vi "MES_Post.vi"(8 "error in (no error)":errorcluster, 10 "Body":string, 11 "Path":string) -> (0 "error out":errorcluster, 1 "Response":string, 2 "Code":string, 3 "MES OK":bool)   [LabVIEW 2018]
uses:
  <vilib>/httpClient/LabVIEWHTTPClient.lvlib
  <vilib>/httpClient/POSTBuffer.vi
  <vilib>/regexp/Match Regular Expression.xnode
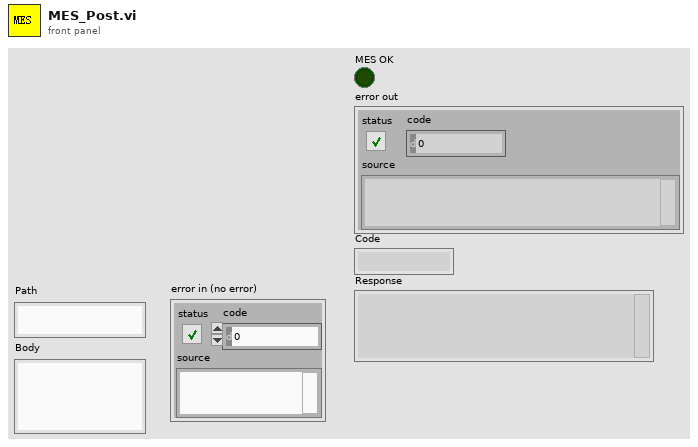
[diagram p1: front panel]
types:
  T1 = typedef "LabVIEWHTTPClient.lvlib/ClientHandle.ctl" = refnum<k1>
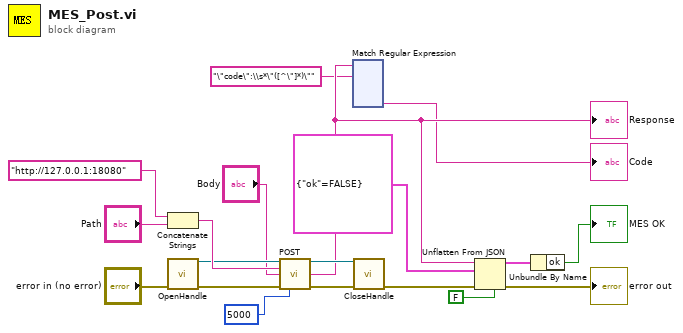
[diagram p0: block diagram]
diagram:
  n1 = Concatenate Strings("http://127.0.0.1:18080" ("string"), "Path") -> (w13:string)
  n2 = call <vilib>:"OpenHandle.vi"("error in (no error)"="error in (no error)") -> ("client handle out"=w11:T1, "error out"=w14:errorcluster)  [unwired: 13 in]
  n3 = call-poly <vilib>:"POST.vi"("client handle"=w11, "url"=w13, "buffer"="Body", "error in (no error)"=w14, "timeout (10000)"=5000) -> ("client handle out"=w17:T1, "body"=w4:string, "error out"=w16:errorcluster)  [unwired: 7 in, 1 out]
  "Response" <- w4
  n4 = xnode "Match Regular Expression"("input string"=w4, "regular expression"="\"code\":\\s*\"([^\"]*)\"") -> ("submatch 1"=→"Code":string)  [unwired: 4 in, 5 out]
  n5 = call <vilib>:"CloseHandle.vi"("client handle"=w17, "error in (no error)"=w16) -> ("error out"=w8:errorcluster)  [unwired: 13 in]
  n6 = Unflatten From JSON(JSON string=w4, type and defaults=cluster{"ok":bool} {"ok"=FALSE}, strict validation? (F)=FALSE, error in (no error)=w8) -> (value=w7:cluster{"ok":bool}, error out=→"error out":errorcluster)  [unwired: 3 in]
  n7 = Unbundle By Name(w7) -> ("ok"=→"MES OK":bool)
